vi "SPARK Get Basic Config.vi"   [LabVIEW 2027]
doc: "Get the configured basic settings of the SPARK."
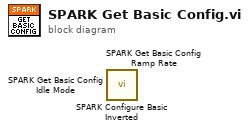
[diagram p0: block diagram]
diagram:
  n1 = call <vilib>:"SPARK Configure Basic Inverted.vi"() -> ()  [unwired: 10 in, 2 out]
  n2 = call <vilib>:"SPARK Get Basic Config Ramp Rate.vi"() -> ()  [unwired: 9 in, 3 out]
  n3 = call <vilib>:"SPARK Get Basic Config Idle Mode.vi"() -> ()  [unwired: 9 in, 3 out]
